vi "Send TurnTable Angle Response.vi"(8 "error in (no error)":errorcluster caption="에러 입력(에러 없음)", 9 "Current Angle":dbl, 10 "id":string, 11 "Instrument Manager 입력":refnum<class "Instrument Manager.lvclass">) -> (0 "error out":errorcluster caption="에러 출력", 3 "Instrument Manager 출력":refnum<class "Instrument Manager.lvclass">)   [LabVIEW 2023, in "Instrument Manager.lvclass"]
uses:
  Instrument Manager.lvclass
  Instrument Manager.lvclass/Instrument Manager.ctl
  TurnTable Angle Response.ctl
  Error Response.ctl
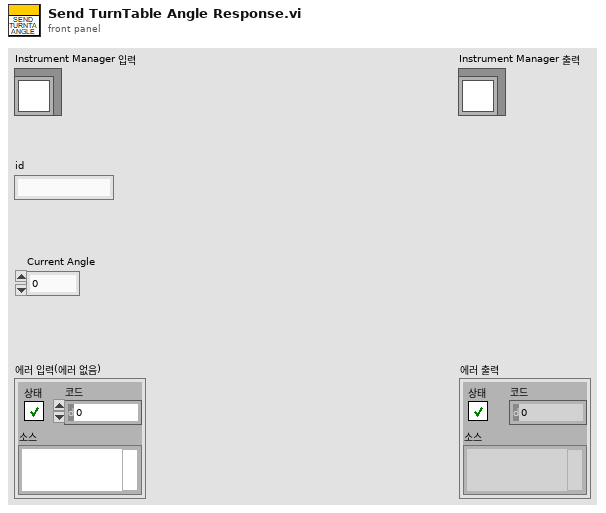
[diagram p1: front panel]
types:
  T1 = typedef "Instrument Manager.lvclass/TurnTable Angle Response.ctl" = cluster{"type":string, "id":string, "status":string, "Result":cluster{"Current Angle":dbl}}
  T2 = cluster{"Reader Q":refnum<queue>, "Writer Q":refnum<queue>}
  T3 = typedef "Instrument Manager.lvclass/Error Response.ctl" = cluster{"type":string, "id":string, "status":string, "error out":errorcluster}
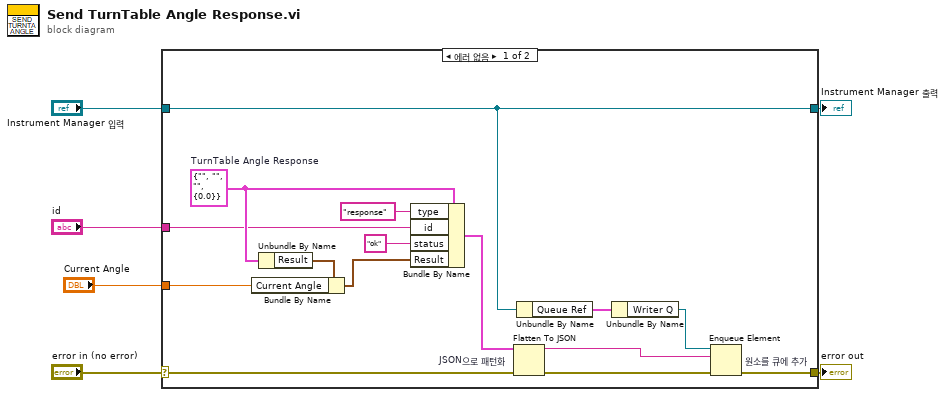
[diagram p0: block diagram]
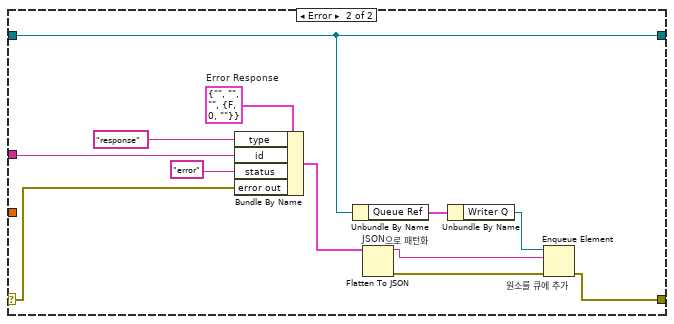
[diagram p2: hidden frame]
diagram:
  n1 = case shown="에러 없음" "error in (no error)" {
    selector: "error in (no error)" -> [w12 w23]
    tunnel: [w7 w25] -> w4
    tunnel: "Instrument Manager 입력" -> [w7 w25]
    tunnel: "Current Angle" -> [w9 _]
    tunnel: "id" -> [w8 w22]
    tunnel: [w10 w24] -> w1
    frame No Error {
      w13 = T1 {"type"="", "id"="", "status"="", "Result"={"Current Angle"=0.0}}  # TurnTable Angle Response
      n2 = Unbundle By Name(w13) -> ("Result"=w19:cluster{"Current Angle":dbl})
      n3 = Bundle By Name(cluster=w19, "Current Angle"=w9) -> (w18:cluster{"Current Angle":dbl})
      n4 = Bundle By Name(cluster=w13, "type"="response", "id"=w8, "status"="ok", "Result"=w18) -> (w17:T1)
      n5 = Flatten To JSON "JSON으로 패턴화"(anything=w17, error in (no error)=w12) -> (JSON string=w14:string, 11:w11:errorcluster)  [unwired: 1 in]
      n6 = Unbundle By Name(w7) -> ("Queue Ref"=w16:T2)
      n7 = Unbundle By Name(w16) -> ("Writer Q"=w15:refnum<queue>)
      n8 = Enqueue Element "원소를 큐에 추가"(queue=w15, element=w14, error in (no error)=w11) -> (error out=w10:errorcluster)  [unwired: 1 in, 2 out]
    }
    frame Error {
      w33 = T3 {"type"="", "id"="", "status"="", "error out"={"status"=FALSE, "code"=0, "source"=""}}  # Error Response
      n9 = Bundle By Name(cluster=w33, "type"="response", "id"=w22, "status"="error", "error out"=w23) -> (w29:T3)
      n10 = Unbundle By Name(w25) -> ("Queue Ref"=w27:T2)
      n11 = Flatten To JSON "JSON으로 패턴화"(anything=w29) -> (JSON string=w32:string, 11:w28:errorcluster)  [unwired: 2 in]
      n12 = Unbundle By Name(w27) -> ("Writer Q"=w26:refnum<queue>)
      n13 = Enqueue Element "원소를 큐에 추가"(queue=w26, element=w32, error in (no error)=w28) -> (error out=w24:errorcluster)  [unwired: 1 in, 2 out]
    }
  }
  "error out" <- w1
  "Instrument Manager 출력" <- w4
